vi "start_recovery_imaging_subvi__684e5953b9.vi"(4 "interval between images (s)":dbl=0.01, 6 "Total number of images to be acquired":i32=1000, 7 "Stop in":bool, 8 "shear cessation point":dbl, 9 "Exposure (s)":dbl=0.0001, 10 "Pulses to start":u32, 11 "Loop Time (ms)":u32=10) -> (1 "array":cluster{dbl, dbl}[](array[cluster]), 2 "task done?":bool, 3 "ReceivedCounts":u32)   [LabVIEW 2023]
uses:
  <vilib>/Utility/error.llb/DialogType.ctl
  <vilib>/DAQmx/write.llb/DAQmx Write (Counter 1D Time 1Chan NSamp).vi
  <vilib>/DAQmx/create/channels.llb/DAQmx Create Channel (CO-Pulse Generation-Time).vi
  <vilib>/DAQmx/configure/timing.llb/DAQmx Timing (Implicit).vi
  <vilib>/DAQmx/create/channels.llb/DAQmx Create Channel (CI-Count Edges).vi
  <vilib>/DAQmx/miscellaneous.llb/DAQmx Fill In Error Info.vi
  <resource>/objmgr/daqmx.rc
  <vilib>/DAQmx/read.llb/DAQmx Read (Counter DBL 1Chan 1Samp).vi
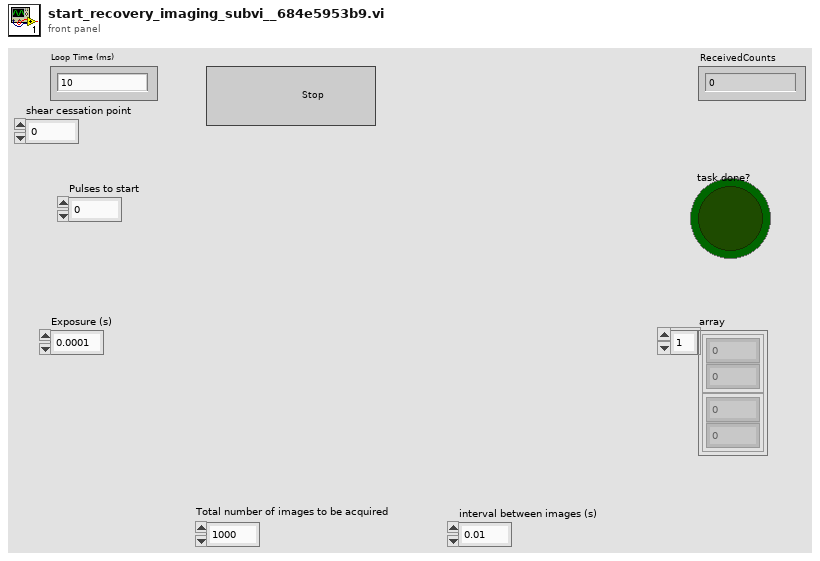
[diagram p1: front panel]
types:
  T1 = typedef "DialogType.ctl" = u16
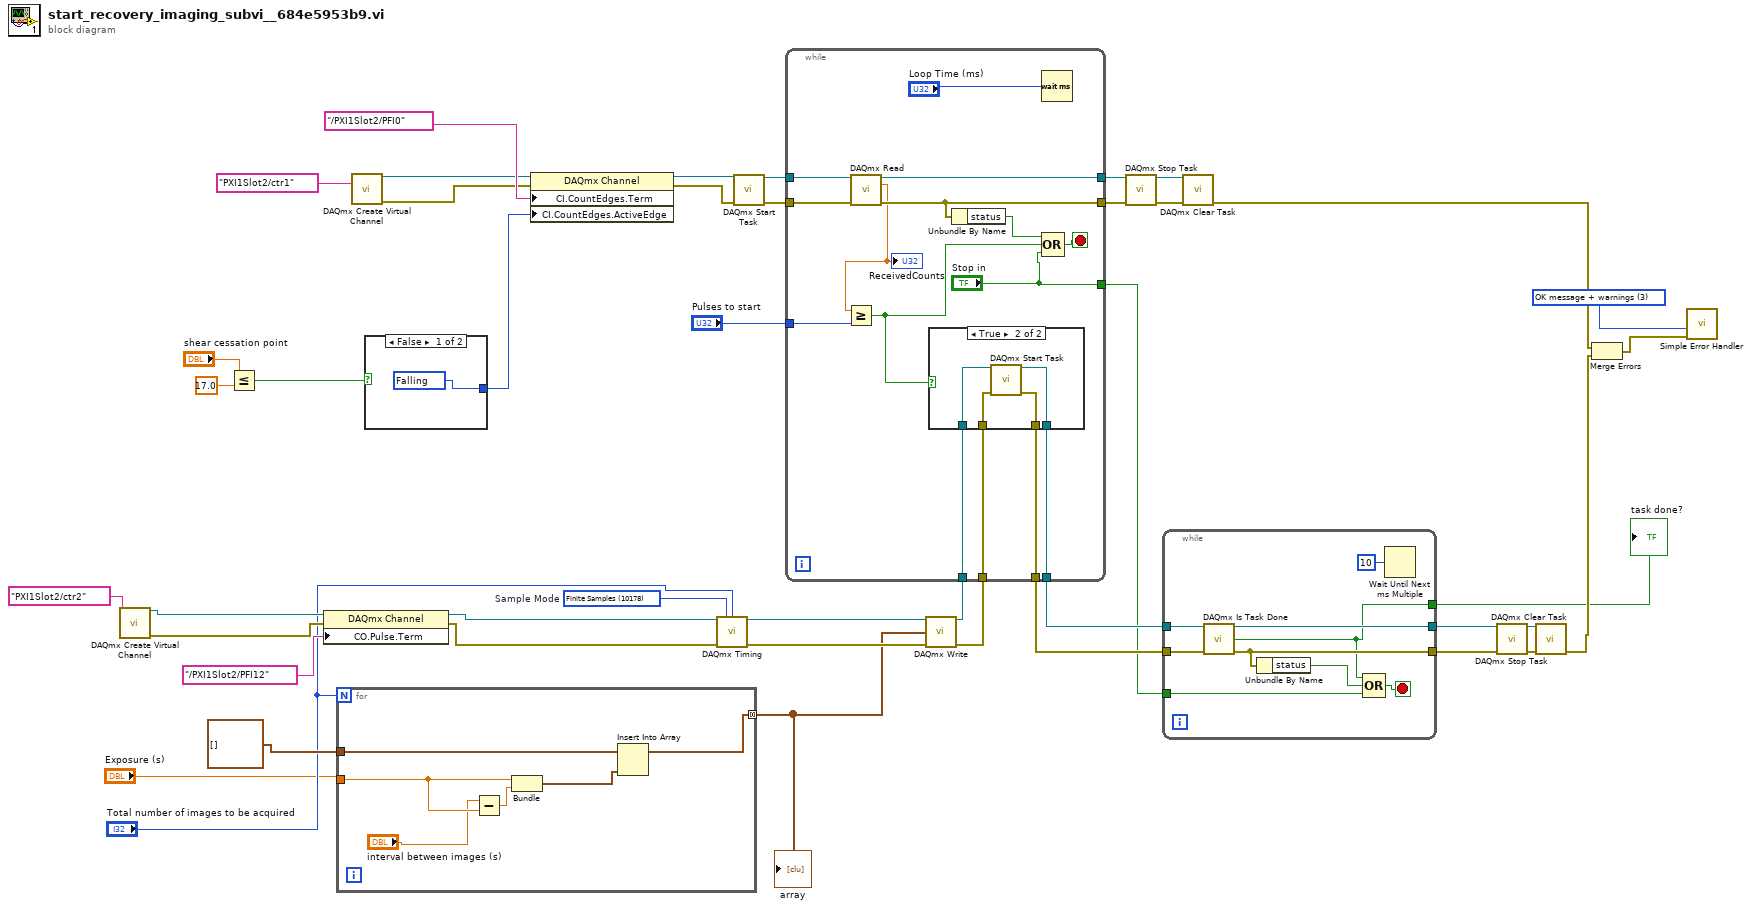
[diagram p0: block diagram]
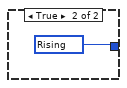
[diagram p2: hidden frame]
diagram:
  w22 = 10178 items=["Finite Samples"=10178, "Continuous Samples"=10123, "Hardware Timed Single Point"=12522]  # Sample Mode
  w27 = T1 3 items=["no dialog", "OK message", "continue or stop message", "OK message + warnings", "continue/stop + warnings"] ("type of dialog (OK msg:1)")
  n1 = call-poly <vilib>:"DAQmx Create Virtual Channel.vi"("counter"=tag "PXI1Slot2/ctr2") -> ("task out"=w21:refnum<k21>, "error out"=w20:errorcluster)  [unwired: 13 in]
  n2 = Less Or Equal?(x="shear cessation point", y=17.0) -> (x <= y?=w2:bool)
  n3 = property class="DAQmx Channel"(reference=w21, error in=w20, "CO.Pulse.Term"=tag "/PXI1Slot2/PFI12") -> (reference out=w26:refnum<k21>, error out=w25:errorcluster)
  n4 = for {
    N: "Total number of images to be acquired" -> [_]
    tunnel: [w50] -> w24 mode=concatenating
    tunnel: "Exposure (s)" -> [w47]
    tunnel: cluster{dbl, dbl}[] [] ("array") -> [w45]
    n5 = Subtract(x="interval between images (s)", y=w47) -> (x-y=w48:dbl)
    n6 = Bundle("Exposure (s)"=w47, w48) -> (w49:cluster{"Exposure (s)":dbl, dbl})  [unwired: 1 in]
    n7 = Insert Into Array(array=w45, new element=w49) -> (w50:cluster{dbl, dbl}[])  [unwired: 1 in]
  }
  "array" <- w24
  n8 = call-poly <vilib>:"DAQmx Create Virtual Channel.vi"("counter"=tag "PXI1Slot2/ctr1") -> ("task out"=w7:refnum<k21>, "error out"=w8:errorcluster)  [unwired: 13 in]
  n9 = case shown="False" w2 {
    tunnel: [w51 w52] -> w1
    frame False {
      w51 = 10171 items=["Rising"=10280, "Falling"=10171] ("CI.CountEdges.ActiveEdge")
    }
    frame True {
      w52 = 10280 items=["Rising"=10280, "Falling"=10171] ("CI.CountEdges.ActiveEdge")
    }
  }
  n10 = property class="DAQmx Channel"(reference=w7, error in=w8, "CI.CountEdges.Term"=tag "/PXI1Slot2/PFI0", "CI.CountEdges.ActiveEdge"=w1) -> (reference out=w10:refnum<k21>, error out=w9:errorcluster)
  n11 = call-poly <vilib>:"DAQmx Timing.vi"("task/channels in"=w26, "sample mode"=w22, "samples per channel"="Total number of images to be acquired", "error in"=w25) -> ("task out"=w30:refnum<k21>, "error out"=w31:errorcluster)  [unwired: 10 in]
  n12 = call <vilib>:"DAQmx Start Task.vi"("task/channels in"=w10, "error in"=w9) -> ("task out"=w5:refnum<k21>, "error out"=w6:errorcluster)  [unwired: 12 in]
  n13 = call-poly <vilib>:"DAQmx Write.vi"("task/channels in"=w30, "data"=w24, "error in"=w31) -> ("task out"=w40:refnum<k21>, "error out"=w41:errorcluster)  [unwired: 10 in, 1 out]
  n14 = while {
    tunnel: w5 -> [w67]
    tunnel: w6 -> [w66]
    tunnel: [w64] -> w12
    tunnel: [w65] -> w11
    tunnel: ["Stop in"] -> w36
    tunnel: "Pulses to start" -> [w57]
    tunnel: w40 -> [w56]
    tunnel: w41 -> [w55]
    tunnel: [w54] -> w42
    tunnel: [w53] -> w43
    stop <- w58 stop-if-true
    n15 = call-poly <vilib>:"DAQmx Read.vi"("task/channels in"=w67, "error in"=w66) -> ("task out"=w65:refnum<k21>, "data"=w62:dbl, "error out"=w64:errorcluster)  [unwired: 11 in]
    "ReceivedCounts" <- w62
    n16 = Greater Or Equal?(x=w62, y=w57) -> (x >= y?=w59:bool)
    n17 = case shown="True" w59 {
      tunnel: w56 -> [_ w71]
      tunnel: w55 -> [_ w68]
      tunnel: [_ w70] -> w53
      tunnel: [_ w69] -> w54
      frame False {
      }
      frame True {
        n18 = call <vilib>:"DAQmx Start Task.vi"("task/channels in"=w71, "error in"=w68) -> ("task out"=w70:refnum<k21>, "error out"=w69:errorcluster)  [unwired: 12 in]
      }
    }
    n19 = Unbundle By Name(w64) -> ("status"=w61:bool)
    n20 = Wait (ms)(milliseconds to wait="Loop Time (ms)") -> ()  [unwired: 1 out]
    n21 = Compound Arithmetic op=OR(w61, w59, "Stop in") -> (w58:bool)
  }
  n22 = call <vilib>:"DAQmx Stop Task.vi"("task/channels in"=w11, "error in"=w12) -> ("task out"=w14:refnum<k21>, "error out"=w13:errorcluster)  [unwired: 12 in]
  n23 = while {
    tunnel: w42 -> [w80]
    tunnel: [w77] -> w17
    tunnel: [w78] -> w18
    tunnel: w43 -> [w72]
    tunnel: [w74] -> w32
    tunnel: w36 -> [w73]
    stop <- w79 stop-if-true
    n24 = call <vilib>:"DAQmx Is Task Done.vi"("task/channels in"=w72, "error in"=w80) -> ("task out"=w78:refnum<k21>, "task done?"=w74:bool, "error out"=w77:errorcluster)  [unwired: 11 in]
    n25 = Unbundle By Name(w77) -> ("status"=w76:bool)
    n26 = Compound Arithmetic op=OR(w74, w76, w73) -> (w79:bool)
    n27 = Wait Until Next ms Multiple(millisecond multiple=u32 10) -> ()  [unwired: 1 out]
  }
  "task done?" <- w32
  n28 = call <vilib>:"DAQmx Clear Task.vi"("task in"=w14, "error in"=w13) -> ("error out"=w39:errorcluster)  [unwired: 13 in]
  n29 = call <vilib>:"DAQmx Stop Task.vi"("task/channels in"=w18, "error in"=w17) -> ("task out"=w29:refnum<k21>, "error out"=w28:errorcluster)  [unwired: 12 in]
  n30 = call <vilib>:"DAQmx Clear Task.vi"("task in"=w29, "error in"=w28) -> ("error out"=w38:errorcluster)  [unwired: 13 in]
  n31 = Merge Errors(w39, w38) -> (w37:errorcluster)
  n32 = call <vilib>:"Simple Error Handler.vi"("type of dialog (OK msg:1)"=w27, "error in (no error)"=w37) -> ()  [unwired: 3 in, 5 out]
